vi "Scale Double R16.vi"(0 "x":dbl, 1 "factor":dbl) -> (2 "y":dbl)   [LabVIEW 2026]
doc: "Round16 gRPC-loop proof: y = x * factor, authored as AIXML, compiled through NI's gRPC ConvertAIXMLToVI, and run through RunVIAndReadValues. Demonstrates the canonical AI -> VI -> run pipeline that was dead in the 2018-only station and is restored in this 2026-capable session. All three terminals carry conIdx so the VI is also Callable (LV014)."
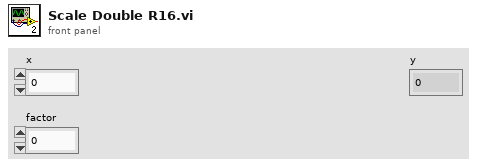
[diagram p1: front panel]
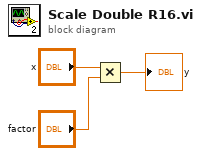
[diagram p0: block diagram]
diagram:
  n1 = Multiply(x="x", y="factor") -> (x*y=→"y":dbl)
